vi "GOOP_ApplyOverlayIcon.vi"(8 "error in (no error)":errorcluster, 10 "IconName(NoPngExtension)":string, 11 "Object":u64) -> (0 "error out":errorcluster)   [LabVIEW 2020]
uses:
  <resource>/Framework/Providers/API/mxLvOverlayState.ctl
  <resource>/Framework/Providers/API/mxLvOverlayAlias.ctl
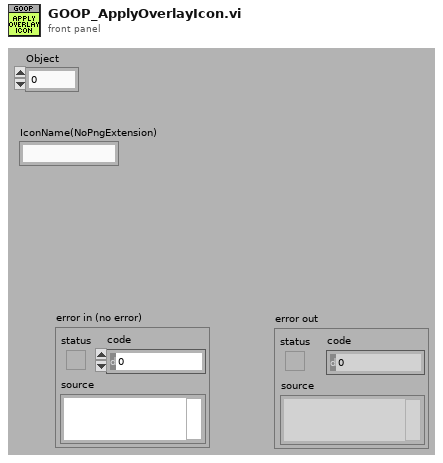
[diagram p1: front panel]
types:
  T1 = typedef "mxLvOverlayAlias.ctl" = cluster{"Overlay Alias":string, "Icon File Name":path}
  T2 = typedef "mxLvOverlayState.ctl" = cluster{"Overlay Alias":string, "Active":bool}
  T3 = typedef "ItemRef.ctl" = u64
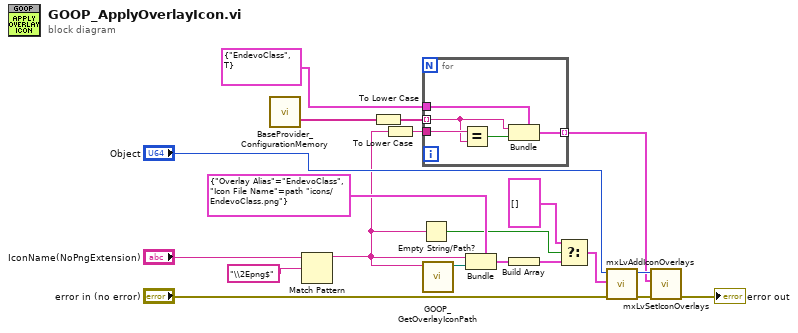
[diagram p0: block diagram]
diagram:
  n1 = call "BaseProvider_ConfigurationMemory.vi"() -> ("ClassItemIconNames"=w11:string[])  [unwired: 13 in, 6 out]
  n2 = Match Pattern(string="IconName(NoPngExtension)", regular expression="\\2Epng$" ("string")) -> (before substring=w1:string)  [unwired: 1 in, 3 out]
  n3 = To Lower Case(string=w11) -> (all lower case string=w4:string[])
  n4 = To Lower Case(string=w1) -> (all lower case string=w5:string)
  n5 = Empty String/Path?(string/path=w1) -> (empty?=w10:bool)
  n6 = for {
    tunnel: w5 -> [w25]
    tunnel: T2 {"Overlay Alias"="EndevoClass", "Active"=TRUE} ("Icon Overlay State") -> [w23]
    tunnel: [w22] -> w12 mode=indexing
    tunnel: w4 -> [w21] mode=indexing
    n7 = Equal?(x=w25, y=w21) -> (x = y?=w24:bool)
    n8 = Bundle(cluster=w23, "Overlay Alias"=w21, "Active"=w24) -> (w22:T2)
  }
  n9 = call "GOOP_GetOverlayIconPath.vi"("IconName(NoPngExtension)"=w1) -> ("IconPath"=w20:path)  [unwired: 10 in]
  n10 = Bundle(cluster=T1 {"Overlay Alias"="EndevoClass", "Icon File Name"=path "icons/EndevoClass.png"} ("Icon Overlay Alias"), "Overlay Alias"=w1, "Icon File Name"=w20) -> (w19:T1)
  n11 = Build Array(w19) -> (w9:T1[])
  n12 = Select(t=T1[] [], s=w10, f=w9) -> (s? t:f=w8:T1[])
  n13 = call <resource>:"mxLvAddIconOverlays.vi"("error in"="error in (no error)", "Overlay Aliases"=w8, "Item"="Object") -> ("error out"=w16:errorcluster, "Item"=w17:T3)  [unwired: 7 in]
  n14 = call <resource>:"mxLvSetIconOverlays.vi"("error in"=w16, "Overlay States"=w12, "Item"=w17) -> ("error out"=→"error out":errorcluster)  [unwired: 7 in, 1 out]
